vi "DMM Read DC Volts Stats.vi"(0 "instrument handle":refnum<k15>, 5 "Number of Readings":i32=10, 11 "error in":errorcluster) -> (4 "instrument handle out":refnum<k15>, 6 "Mean (V)":dbl, 8 "Std Dev (V)":dbl, 15 "error out":errorcluster)   [LabVIEW 2026]
doc: "Configures the NI-DMM session for DC volts on the 10 V range with 6.5 digits and an input resistance above 10 GOhm (the cell is not loaded), takes Number of Readings readings with niDMM Read Multi Point and returns their mean and sample standard deviation. Does not open or close the session. An incoming error skips the measurement."
uses:
  <vilib>/Analysis/NI_AALBase.lvlib
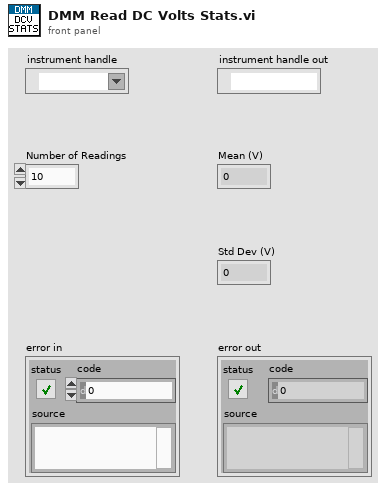
[diagram p1: front panel]
types:
  T1 = enum16{"Immediate", "External", "TTL 0", "TTL 1", "TTL 2", "TTL 3", "TTL 4", "TTL 5", "TTL 6", "Interval", "Software", "TTL 7", "PXI Star", "LBR Trig 1", "Aux Trig 1"}
  T2 = enum16{"DC Volts", "AC Volts", "DC Current", "AC Current", "2-wire Resistance", "4-wire Resistance", "Diode", "Frequency", "Period", "AC Volts DC Coupled", "Capacitance", "Inductance", "Temperature"}
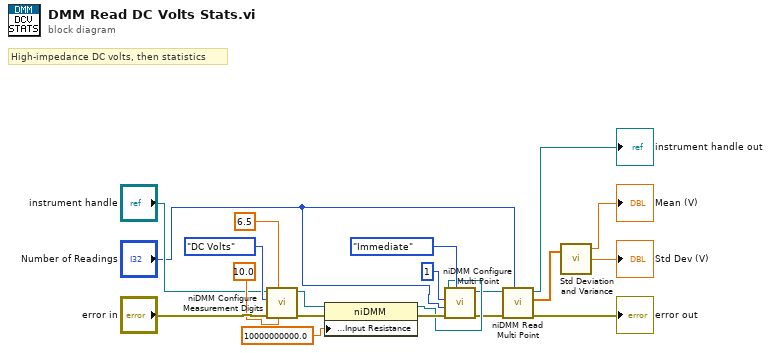
[diagram p0: block diagram]
diagram:
  # "High-impedance DC volts, then statistics"
  n1 = call <instrlib>:"niDMM Configure Measurement Digits.vi"("Range"=10.0, "Resolution in Digits"=6.5, "error in (no error)"="error in", "Function"=T2."DC Volts", "instrument handle"="instrument handle") -> ("error out"=w14:errorcluster, "instrument handle out"=w15:refnum<k15>)  [unwired: 5 in]
  n2 = property class="niDMM"(reference=w15, error in=w14, "Configuration:Measurement Options:Input Resistance"=10000000000.0 ("Input Resistance")) -> (reference out=w9:refnum<k15>, error out=w12:errorcluster)
  n3 = call <instrlib>:"niDMM Configure Multi Point.vi"("Sample Trigger"=T1."Immediate", "error in (no error)"=w12, "Sample Count"="Number of Readings", "Trigger Count"=1, "instrument handle"=w9) -> ("error out"=w8:errorcluster, "instrument handle out"=w6:refnum<k15>)  [unwired: 5 in]
  n4 = call <instrlib>:"niDMM Read Multi Point.vi"("Number to Read"="Number of Readings", "error in (no error)"=w8, "instrument handle"=w6) -> ("error out"=→"error out":errorcluster, "Measurements"=w5:dbl[], "instrument handle out"=→"instrument handle out":refnum<k15>)  [unwired: 5 in, 1 out]
  n5 = call <vilib>:"Std Deviation and Variance.vi"("X"=w5) -> ("mean"=→"Mean (V)":dbl, "standard deviation"=→"Std Dev (V)":dbl)  [unwired: 1 in, 1 out]
